vi "test security.vi"() -> ()   [LabVIEW 2019]
uses:
  <userlib>/_OpenG.lib/md5/md5.llb/MD5 Message Digest (Hexadecimal String)__ogtk.vi
  <vilib>/httpClient/POSTBuffer.vi
  <vilib>/httpClient/LabVIEWHTTPClient.lvlib
panel:
  out "x .and. y?":bool
  out "body":string
  out "MD5 Message Digest":string
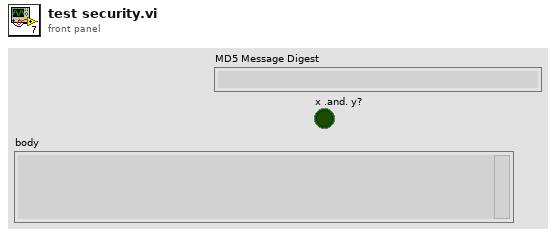
[diagram p1: front panel]
types:
  T1 = cluster{"action":string, "username":string, "password":string}
  T2 = cluster{"status":string, "data":cluster{"id":string, "username":string, "password":string, "delete":string}[]}
  T3 = typedef "LabVIEWHTTPClient.lvlib/ClientHandle.ctl" = refnum<k1>
  T4 = cluster{"id":string, "username":string, "password":string, "delete":string}[]
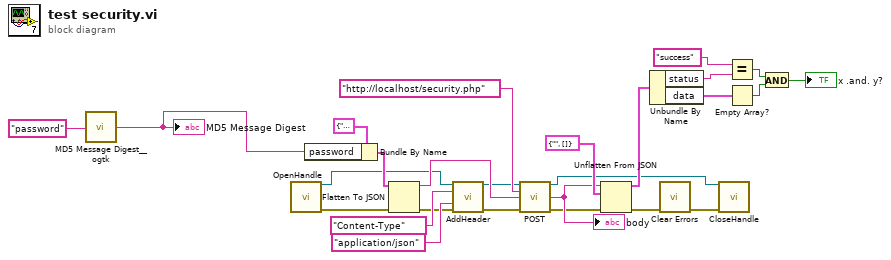
[diagram p0: block diagram]
diagram:
  n1 = call-poly <userlib>:"MD5 Message Digest__ogtk.vi"("Message"="password") -> ("MD5 Message Digest"=w2:string)
  "MD5 Message Digest" <- w2
  n2 = call <vilib>:"OpenHandle.vi"() -> ("client handle out"=w5:T3, "error out"=w4:errorcluster)  [unwired: 14 in]
  n3 = Bundle By Name(cluster=T1 {"action"="read", "username"="geologic", "password"=""}, "password"=w2) -> (w13:T1)
  n4 = Flatten To JSON(anything=w13, error in (no error)=w4) -> (JSON string=w23:string, 11:w16:errorcluster)  [unwired: 1 in]
  n5 = call <vilib>:"AddHeader.vi"("client handle"=w5, "header"="Content-Type", "value"="application/json", "error in (no error)"=w16) -> ("client handle out"=w19:T3, "error out"=w18:errorcluster)  [unwired: 10 in]
  n6 = call-poly <vilib>:"POST.vi"("client handle"=w19, "url"="http://localhost/security.php", "buffer"=w23, "error in (no error)"=w18) -> ("client handle out"=w6:T3, "body"=w17:string, "error out"=w15:errorcluster)  [unwired: 8 in, 1 out]
  "body" <- w17
  n7 = Unflatten From JSON(JSON string=w17, type and defaults=T2 {"status"="", "data"=[]}, error in (no error)=w15) -> (value=w24:T2, error out=w14:errorcluster)  [unwired: 4 in]
  n8 = Unbundle By Name(w24) -> ("status"=w11:string, "data"=w12:T4)
  n9 = call <vilib>:"Clear Errors.vi"("error in (no error)"=w14) -> ("error out"=w7:errorcluster)  [unwired: 5 in, 1 out]
  n10 = call <vilib>:"CloseHandle.vi"("client handle"=w6, "error in (no error)"=w7) -> ()  [unwired: 13 in, 1 out]
  n11 = Equal?(x="success", y=w11) -> (x = y?=w9:bool)
  n12 = Empty Array?(array=w12) -> (empty?=w8:bool)
  n13 = And(x=w9, y=w8) -> (x .and. y?=→"x .and. y?":bool)
